vi "VM Spy - Dialog - Create variable.vi"(11 "VC Handle":T1=-1) -> (0 "OK out":bool, 1 "writer ID out":u32, 2 "var name":string)   [LabVIEW 2021]
doc: "::: CalcExpress Toolkit :::\nCopyright (c) 2000-2026 Konstantin Shifershteyn. All rights reserved."
uses:
  vi.lib/addons/CalcExpress/cetypes.llb/VarMan Variable Context Handle.ctl
  vi.lib/addons/CalcExpress/cetypes.llb/CalcExpress Data Type.ctl
panel:
  in  "writer ID":u32
  in  "assign value":bool
  in  "cancel":bool
  in  "ok":bool
  in  "Data type":u32(ring)=1 items=["DBL Number"=1, "1D Array of DBL"=3, "2D Array of DBL"=4, "CDB Number"=5, "1D Array of CDB"=6, "2D Array of CDB"=7, "String"=0, "1D Array of String"=8, "2D Array of String"=9, "Index Range"=252]
  in  "Variable name":string
  out "Context":string
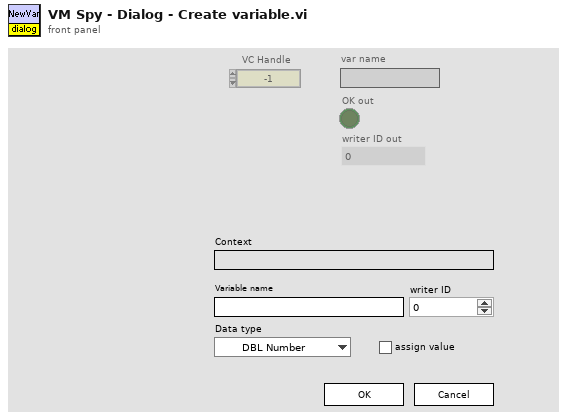
[diagram p1: front panel]
types:
  T1 = typedef "VarMan Variable Context Handle.ctl" = i32
  T2 = typedef "eventvkey.ctl" = enum16{"ASCII", "Enter", "Return", "Shift", "Ctrl", "Alt", "Cmd", "Opt", "Caps", "NumLock", "Clear", "Break", "Up", "Down", "Left", "Right", "Insert", "Delete", "Home", "End", "PageUp", "PageDown", "Escape", "Help", "Pause", "ScrollLock", "F1", "F2", "F3", "F4", "F5", "F6", "F7", "F8", "F9", "F10", "F11", "F12", "F13", "F14", "F15", "F16", "F17", "F18", "F19", "F20", "F21", "F22", "F23", "F24", "Play", "VolumeUp", "VolumeDown", "Mute", "Two Byte Char"}
  T3 = cluster{"Shift":bool, "Ctrl":bool, "Alt":bool, "Cmd":bool, "Opt":bool}
  T4 = typedef "CalcExpress Data Type.ctl" = enum32{"String", "DBL Number", "identifier", "1D Array of DBL", "2D Array of DBL", "CDB Number", "1D Array of CDB", "2D Array of CDB", "1D Array of String", "2D Array of String", "Unknown data type"}
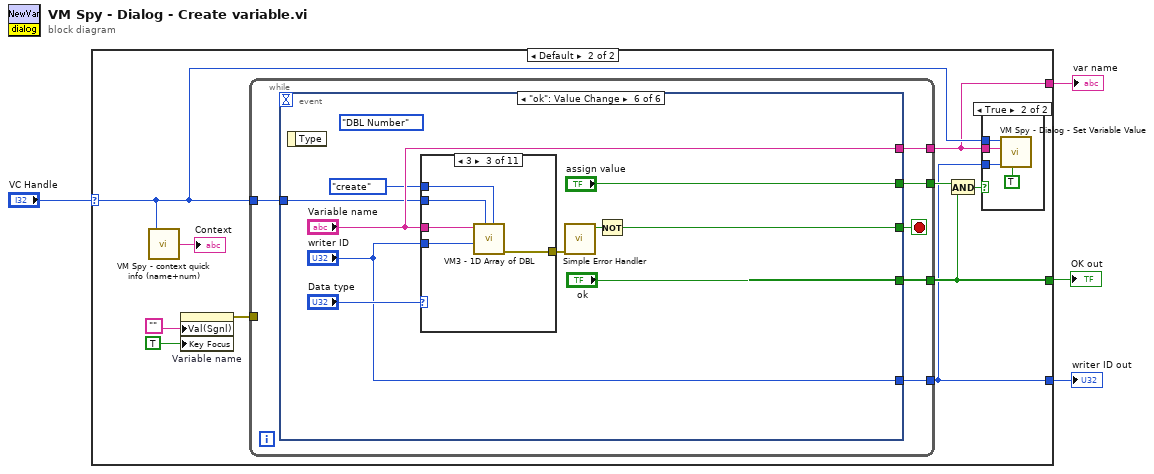
[diagram p0: block diagram]
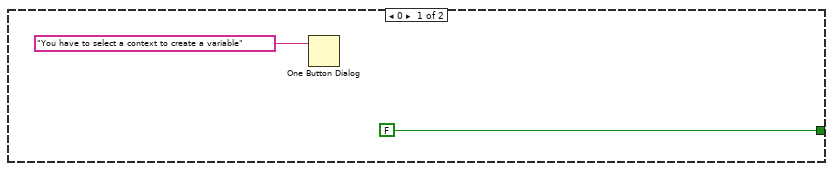
[diagram p2: hidden frame]
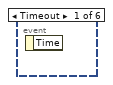
[diagram p3: hidden frame]
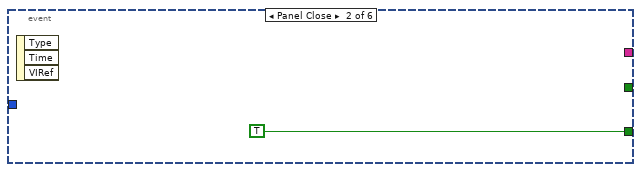
[diagram p4: hidden frame]
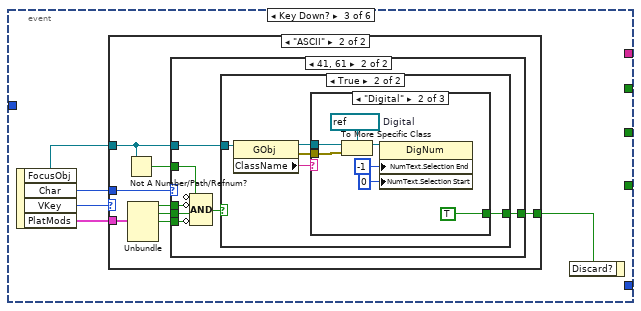
[diagram p5: hidden frame]
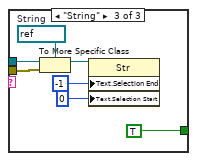
[diagram p10: hidden frame]
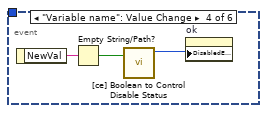
[diagram p11: hidden frame]
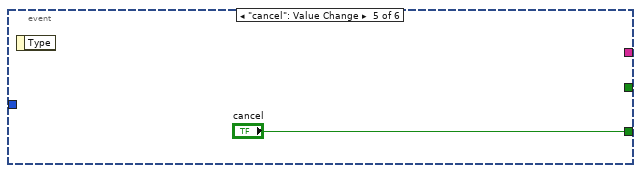
[diagram p12: hidden frame]
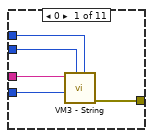
[diagram p13: hidden frame]
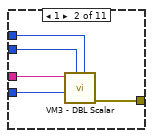
[diagram p14: hidden frame]
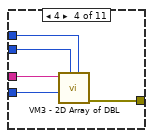
[diagram p15: hidden frame]
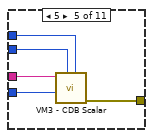
[diagram p16: hidden frame]
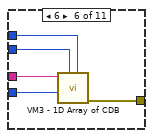
[diagram p17: hidden frame]
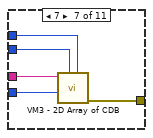
[diagram p18: hidden frame]
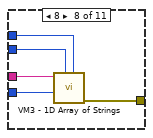
[diagram p19: hidden frame]
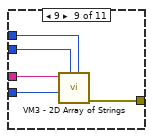
[diagram p20: hidden frame]
diagram:
  n1 = case shown="Default" "VC Handle" {
    selector: "VC Handle" -> [_ w12]
    tunnel: [FALSE w14] -> w4
    tunnel: [_ w11] -> w2
    tunnel: [_ w7] -> w1
    frame 0 {
      n2 = One Button Dialog(message="You have to select a context to create a variable") -> ()  [unwired: 1 in, 1 out]
    }
    frame Default {
      n3 = call "VM Spy - context quick info (name+num).vi"("handle"=w12) -> ("context info"=→"Context":string)  [unwired: 4 in]
      n4 = property on="Variable name" class="Str"("Val(Sgnl)"="", "Key Focus"=TRUE) -> (error out=w8:errorcluster)  [unwired: 2 in, 1 out]
      n5 = while {
        tunnel: [w21] -> w14
        tunnel: [w20] -> w11
        tunnel: [w18] -> w13
        tunnel: w12 -> [w19]
        tunnel: w8 -> [_]
        tunnel: [w17] -> w7
        stop <- w22 stop-if-true
        n6 = event shown="[5] \"ok\": Value Change" {
          selector: _ -> [_ _ _ _ _ _]
          dyn-events: _ -> [_ _ _ _ _ _]
          timeout: _ -> [_ _ _ _ _ _]
          tunnel: [_ TRUE _ _ "cancel" w72] -> w22
          tunnel: [_ _ _ _ _ "Variable name"] -> w20
          tunnel: [_ _ _ _ _ "ok"] -> w21
          tunnel: w19 -> [_ _ _ _ _ w70]
          tunnel: [_ _ _ _ _ "assign value"] -> w18
          tunnel: [_ _ _ _ _ "writer ID"] -> w17
          event Timeout {
            n7 = event-data() -> ()  [unwired: 1 in, 1 out]
          }
          event Panel Close {
            n8 = event-data() -> ()  [unwired: 1 in, 3 out]
          }
          event Key Down? {
            n9 = event-data() -> ("FocusObj"=w26:refnum<vi>, "Char"=w27:i16, "VKey"=w28:T2, "PlatMods"=w25:T3)  [unwired: 1 in]
            n10 = case shown="\"ASCII\"" w28 {
              tunnel: w25 -> [_ w36]
              tunnel: [_ w30] -> w24
              tunnel: w27 -> [_ w32]
              tunnel: w26 -> [_ w31]
              frame Default {
              }
              frame "ASCII" {
                n11 = Not A Number/Path/Refnum?(number/path/refnum=w31) -> (NaN/Path/Refnum?=w29:bool)
                n12 = Unbundle(w36) -> ("Shift"=w35:bool, "Ctrl"=w34:bool, "Alt"=w33:bool)  [unwired: 2 out]
                n13 = case shown="41, 61" w32 {
                  tunnel: w35 -> [_ w43]
                  tunnel: w34 -> [_ w42]
                  tunnel: w33 -> [_ w41]
                  tunnel: w31 -> [_ w39]
                  tunnel: [_ w38] -> w30
                  tunnel: w29 -> [_ w37]
                  frame Default {
                  }
                  frame 65, 97 {
                    n14 = Compound Arithmetic op=AND(invert w37, invert w43, w42, invert w41) -> (w40:bool)
                    n15 = case shown="True" w40 {
                      tunnel: w39 -> [_ w48]
                      tunnel: [_ w46] -> w38
                      frame False {
                      }
                      frame True {
                        n16 = property class="GObj"(reference=w48) -> (reference out=w45:refnum<vi>, error out=w44:errorcluster, "ClassName"=w47:string)  [unwired: 1 in]
                        n17 = case shown="\"Digital\"" w47 {
                          tunnel: [_ TRUE TRUE] -> w46
                          tunnel: w45 -> [_ w53 w60]
                          tunnel: w44 -> [_ w52 w59]
                          frame Default {
                          }
                          frame "Digital" {
                            w54 = refnum<vi> refnum  # Digital
                            n18 = To More Specific Class(target class=w54, reference=w53, error in=w52) -> (specific class reference=w51:refnum<vi>)  [unwired: 1 out]
                            n19 = property class="DigNum"(reference=w51, "NumText.Selection End"=-1 ("Numeric Text.Selection:End"), "NumText.Selection Start"=u32 0 ("Numeric Text.Selection:Start")) -> ()  [unwired: 1 in, 2 out]
                          }
                          frame "String" {
                            w61 = refnum<vi> refnum  # String
                            n20 = To More Specific Class(target class=w61, reference=w60, error in=w59) -> (specific class reference=w58:refnum<vi>)  [unwired: 1 out]
                            n21 = property class="Str"(reference=w58, "Text.Selection End"=-1 ("Numeric Text.Selection:End"), "Text.Selection Start"=u32 0 ("Numeric Text.Selection:Start")) -> ()  [unwired: 1 in, 2 out]
                          }
                        }
                      }
                    }
                  }
                }
              }
            }
            n22 = event-data("Discard?"=w24) -> ()  [unwired: 1 in, 1 out]
          }
          event "Variable name": Value Change {
            n23 = event-data() -> ("NewVal"=w65:string)  [unwired: 1 in]
            n24 = Empty String/Path?(string/path=w65) -> (empty?=w64:bool)
            n25 = call "[ce] Boolean to Control Disable Status.vi"("Status in"=w64) -> ("Control Disable if True"=w63:u8)  [unwired: 3 in, 1 out]
            n26 = property on="ok" class="Bool"("DisabledEnum"=w63) -> ()  [unwired: 2 in, 2 out]
          }
          event "cancel": Value Change {
            n27 = event-data() -> ()  [unwired: 1 in, 1 out]
          }
          event "ok": Value Change {
            (unwired) CalcExpress_Data_Type."DBL Number" ("type")
            n28 = event-data() -> ()  [unwired: 1 in, 1 out]
            n29 = case shown="3" "Data type" {
              selector: "Data type" -> [_ _ _ _ _ _ _ _ _ w125 _]
              tunnel: "Variable name" -> [w81 w86 w91 w96 w101 w106 w111 w116 w121 w127 _]
              tunnel: w70 -> [w79 w84 w89 w94 w99 w104 w109 w114 w119 w126 _]
              tunnel: [w80 w85 w90 w95 w100 w105 w110 w115 w120 w128 errorcluster {"status"=TRUE, "code"=7001, "source"=""} ("error out")] -> w74
              tunnel: enum16{"create", "destroy", "write", "read"}."create" ("cmd (read)") -> [w78 w83 w87 w93 w98 w103 w107 w112 w117 w122 _]
              tunnel: "writer ID" -> [w77 w82 w88 w92 w97 w102 w108 w113 w118 w123 _]
              frame 0 {
                n30 = call "VM3 - String.vi"("cmd (read)"=w78, "VC Handle"=w79, "writer ID"=w77, "name_spec"=w81) -> ("error out"=w80:errorcluster)  [unwired: 4 in, 3 out]
              }
              frame 1 {
                n31 = call "VM3 - DBL Scalar.vi"("cmd (read)"=w83, "VC Handle"=w84, "writer ID"=w82, "name_spec"=w86) -> ("error out"=w85:errorcluster)  [unwired: 4 in, 3 out]
              }
              frame 3 {
                n32 = call "VM3 - 1D Array of DBL.vi"("cmd (read)"=w87, "VC Handle"=w89, "writer ID"=w88, "name_spec"=w91) -> ("error out"=w90:errorcluster)  [unwired: 4 in, 3 out]
              }
              frame 4 {
                n33 = call "VM3 - 2D Array of DBL.vi"("cmd (read)"=w93, "VC Handle"=w94, "writer ID"=w92, "name_spec"=w96) -> ("error out"=w95:errorcluster)  [unwired: 4 in, 3 out]
              }
              frame 5 {
                n34 = call "VM3 - CDB Scalar.vi"("cmd (read)"=w98, "VC Handle"=w99, "writer ID"=w97, "name_spec"=w101) -> ("error out"=w100:errorcluster)  [unwired: 4 in, 3 out]
              }
              frame 6 {
                n35 = call "VM3 - 1D Array of CDB.vi"("cmd (read)"=w103, "VC Handle"=w104, "writer ID"=w102, "name_spec"=w106) -> ("error out"=w105:errorcluster)  [unwired: 4 in, 3 out]
              }
              frame 7 {
                n36 = call "VM3 - 2D Array of CDB.vi"("cmd (read)"=w107, "VC Handle"=w109, "writer ID"=w108, "name_spec"=w111) -> ("error out"=w110:errorcluster)  [unwired: 4 in, 3 out]
              }
              frame 8 {
                n37 = call "VM3 - 1D Array of Strings.vi"("cmd (read)"=w112, "VC Handle"=w114, "writer ID"=w113, "name_spec"=w116) -> ("error out"=w115:errorcluster)  [unwired: 4 in, 3 out]
              }
              frame 9 {
                n38 = call "VM3 - 2D Array of Strings.vi"("cmd (read)"=w117, "VC Handle"=w119, "writer ID"=w118, "name_spec"=w121) -> ("error out"=w120:errorcluster)  [unwired: 4 in, 3 out]
              }
              frame 252 {
                n39 = call "[ce] Index Range to Flattened String.vi"() -> ("Flattened string"=w124:string)  [unwired: 11 in]
                n40 = call "VM3 - Arbitrary Data.vi"("cmd (read)"=w122, "var type in"=w125, "VC Handle"=w126, "writer ID"=w123, "flattened value in"=w124, "name_spec"=w127) -> ("error out"=w128:errorcluster)  [unwired: 1 in, 4 out]
              }
              frame 2, 10, Default {
              }
            }
            n41 = call <vilib>:"Simple Error Handler.vi"("error in (no error)"=w74) -> ("error?"=w76:bool)  [unwired: 4 in, 4 out]
            n42 = Not(x=w76) -> (.not. x?=w72:bool)
          }
        }
      }
      n43 = And(x=w13, y=w14) -> (x .and. y?=w15:bool)
      n44 = case shown="True" w15 {
        tunnel: w11 -> [_ w132]
        tunnel: w12 -> [_ w133]
        tunnel: w7 -> [_ w131]
        frame False {
        }
        frame True {
          n45 = call "VM Spy - Dialog - Set Variable Value.vi"("refresh writer ID"=TRUE, "writer ID in"=w131, "var name"=w132, "VC Handle"=w133) -> ()  [unwired: 7 in, 1 out]
        }
      }
    }
  }
  "OK out" <- w4
  "var name" <- w2
  "writer ID out" <- w1
